vi "Read Accounts.vi"(8 "error in":errorcluster, 11 "Accounts File Path":path) -> (0 "error out":errorcluster, 3 "Accounts":T1[](array[typedef]))   [LabVIEW 2026]
doc: "Reads the ATM accounts file (CSV, no header, one record per line: Account Number,First Name,Last Name,Balance) and returns every record as an array of ATM Account clusters. Every field is trimmed of whitespace, Balance is parsed as a number with a period as decimal separator, and empty lines are skipped. An empty Accounts File Path returns error 5001 instead of reading, so no file dialog can ever open. A missing or unreadable file returns the file error and an empty array."
uses:
  <vilib>/Utility/error.llb/Trim Whitespace (string).vi
  <vilib>/Utility/error.llb/Trim Whitespace One-Sided.vi
  Controls/ATM Account.ctl
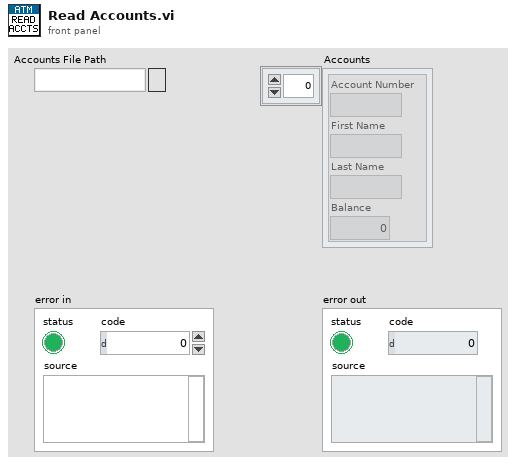
[diagram p1: front panel]
types:
  T1 = typedef "ATM Account.ctl" = cluster{"Account Number":string, "First Name":string, "Last Name":string, "Balance":dbl}
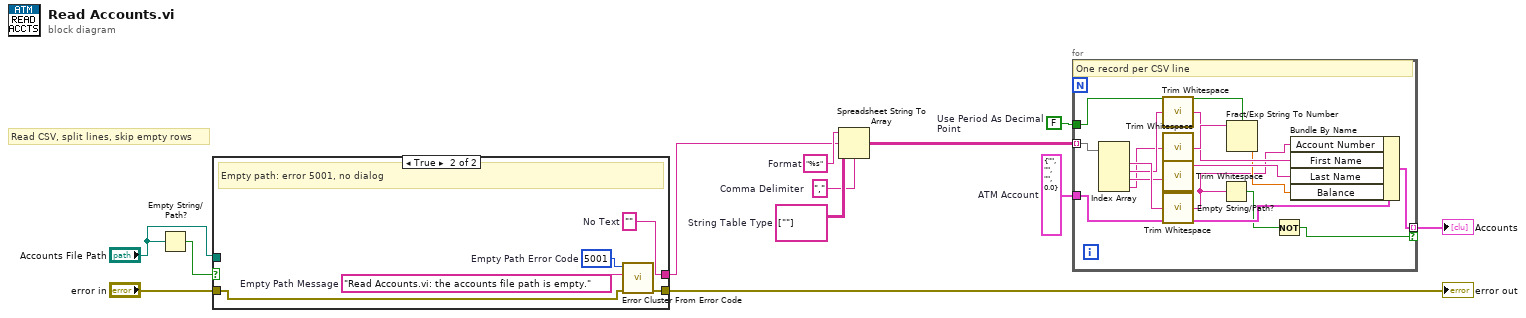
[diagram p0: block diagram]
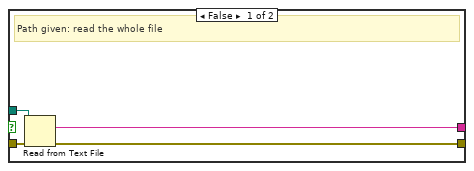
[diagram p2: hidden frame]
diagram:
  w3 = FALSE  # Use Period As Decimal Point
  w4 = T1 {"Account Number"="", "First Name"="", "Last Name"="", "Balance"=0.0}  # ATM Account
  w7 = string[][] [[""]]  # String Table Type
  w6 = ","  # Comma Delimiter
  w9 = "%s"  # Format
  # "Read CSV, split lines, skip empty rows"
  n1 = Empty String/Path?(string/path="Accounts File Path") -> (empty?=w10:bool)
  n2 = case shown="True" w10 {
    tunnel: "Accounts File Path" -> [w16 _]
    tunnel: "error in" -> [w15 w20]
    tunnel: [w14 w18] -> w8
    tunnel: [w13 w17] -> w1
    frame False {
      # "Path given: read the whole file"
      n3 = Read from Text File(file (use dialog)=w16, error in=w15) -> (text=w14:string, error out=w13:errorcluster)  [unwired: 2 in, 2 out]
    }
    frame True {
      w18 = ""  # No Text
      w19 = "Read Accounts.vi: the accounts file path is empty."  # Empty Path Message
      w21 = 5001  # Empty Path Error Code
      # "Empty path: error 5001, no dialog"
      n4 = call <vilib>:"Error Cluster From Error Code.vi"("error in (no error)"=w20, "error message (\"\")"=w19, "error code (0)"=w21) -> ("error out"=w17:errorcluster)  [unwired: 6 in]
    }
  }
  "error out" <- w1
  n5 = Spreadsheet String To Array(delimiter (Tab)=w6, format string=w9, spreadsheet string=w8, array type (2D Dbl)=w7) -> (array=w5:string[][])
  n6 = for {
    tunnel: w5 -> [w36] mode=indexing
    tunnel: w4 -> [w26]
    tunnel: w3 -> [w30]
    tunnel: [w22] -> w2 mode=indexing if=w23
    # "One record per CSV line"
    n7 = Index Array(array=w36) -> (element #1=w35:string, element #2=w34:string, element #3=w33:string, element #4=w32:string)  [unwired: 4 in]
    n8 = call-poly <vilib>:"Trim Whitespace.vi"("string"=w34) -> ("trimmed string"=w29:string)  [unwired: 1 in]
    n9 = call-poly <vilib>:"Trim Whitespace.vi"("string"=w32) -> ("trimmed string"=w31:string)  [unwired: 1 in]
    n10 = call-poly <vilib>:"Trim Whitespace.vi"("string"=w33) -> ("trimmed string"=w28:string)  [unwired: 1 in]
    n11 = call-poly <vilib>:"Trim Whitespace.vi"("string"=w35) -> ("trimmed string"=w25:string)  [unwired: 1 in]
    n12 = Empty String/Path?(string/path=w25) -> (empty?=w24:bool)
    n13 = Fract/Exp String To Number(use system decimal point (T)=w30, string=w31) -> (number=w27:dbl)  [unwired: 2 in, 1 out]
    n14 = Not(x=w24) -> (.not. x?=w23:bool)
    n15 = Bundle By Name(cluster=w26, "Account Number"=w25, "First Name"=w29, "Last Name"=w28, "Balance"=w27) -> (w22:T1)
  }
  "Accounts" <- w2
